vi "Consumer.vi"(8 "error in (no error)":errorcluster, 9 "Data":variant, 10 "Case ID":string, 11 "uService Template in":refnum<class "TCP Writer.lvclass">) -> (0 "error out":errorcluster, 3 "uService Template out":refnum<class "TCP Writer.lvclass">)   [LabVIEW 2020, in "TALOS.lvlib" / "TCP Writer.lvlib" / "TCP Writer.lvclass"]
uses:
  TCP Writer.lvclass
  C:/LabVIEW Code/TALOS/talos/Father of all uServices/Father of all uServices/Father of all uServices.lvclass
  TCP Writer Consumer Case Selector.ctl
  TCP Writer.lvclass/TCP Writer.ctl
  Father of all uServices/Father of all uServices Messages/Consumer Msg/Consumer Msg.lvclass/Consumer Msg.ctl
  Ancestor/Ancestor/Ancestor.lvclass/Ancestor.ctl
  Father of all uServices/Father of all uServices/Father of all uServices.lvclass/Father of all uServices.ctl
  Ancestor/Ancestor/Infinite Message Selector.ctl
  Support VIs/Generate Error.vi
  FGV/Error Memory/Get Error Description.vi
  Ancestor/Ancestor/Read ID.vi
  Support VIs/Get Class Name.vi
  FGV/Error Memory/Error Memory Core.vi
  <vilib>/AdvancedString/Delimited String to 1D String Array.vi
  Support VIs/Circus Root Path.vi
  FGV/Error Memory/Error Crt Lvl checker.vi
  FGV/Error Memory/Error Memory Core.vi/40c8088d-b597-4017-91af-faa98e00292e.vi
  FGV/Error Memory/Error Memory Core.vi/d4a3ab98-063c-4e44-b43d-fbdcfe6c2be2.vi
  Father of all uServices/Father of all uServices/Father of all uServices.lvclass
  C:/LabVIEW Code/TALOS/builds/Actor Framework PPL/Actor Framework.lvlibp/1abvi3w/vi.lib/ActorFramework/Actor/Actor.lvclass
  builds/Actor Framework PPL/Actor Framework.lvlibp/1abvi3w/vi.lib/ActorFramework/Actor/Read Self Enqueuer.vi
  <userlib>/_OpenG.lib/lvdata/lvdata.llb/Get Strings from Enum__ogtk.vi
  builds/Actor Framework PPL/Actor Framework.lvlibp/1abvi3w/vi.lib/ActorFramework/Message Enqueuer/Enqueue.vi
  Support VIs/Global Memory.vi
  Support VIs/Is in Packed Library.vi
  Support VIs/TALOS Root path.vi
  Support VIs/Read CSV worksheet.vi
  Support VIs/Global Constants.vi
  <vilib>/Utility/error.llb/General Error Handler.vi
  Support VIs/Error Log.vi
  Father of all uServices/Father of all uServices Messages/Consumer Msg/Consumer Msg.lvclass
  Ancestor/Ancestor/Ancestor.lvclass
  <vilib>/Comparison/Equal/Equal Functor/Equal Functor.lvclass
  TALOS.lvlib
  C:/LabVIEW Code/TALOS/talos/Ancestor/Ancestor/Ancestor.lvclass
  C:/LabVIEW Code/TALOS/talos/Internal uServices/System uServices/TCP Writer/TCP Writer/TCP Writer.lvclass
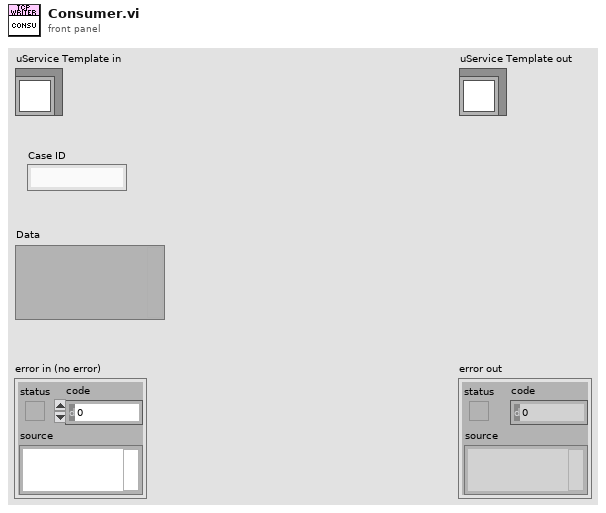
[diagram p1: front panel]
types:
  T1 = typedef "TALOS.lvlib/TCP Writer.lvlib/TCP Writer.lvclass/TCP Writer Consumer Case Selector.ctl" = enum16{"Send message", "Idle", "Check Connection", "Open connection", "Set Client ID"}
  T2 = typedef "TALOS.lvlib/Ancestor.lvlib/Ancestor.lvclass/Infinite Message Selector.ctl" = enum16{"Start", "Stop", "Check", "Flush (Stop all)", "Init"}
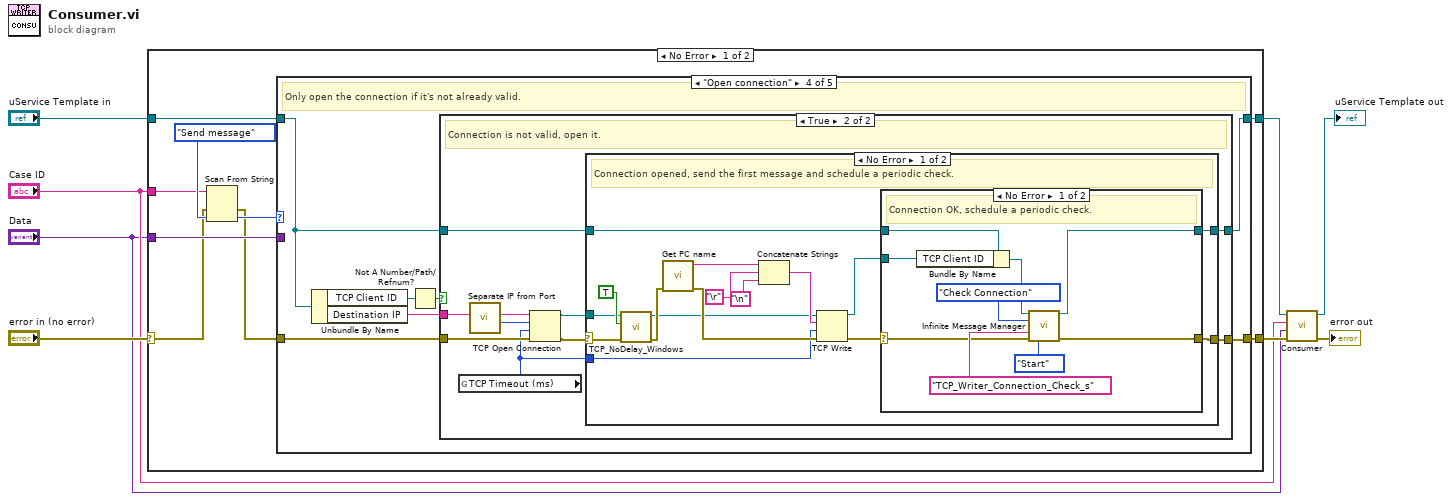
[diagram p0: block diagram]
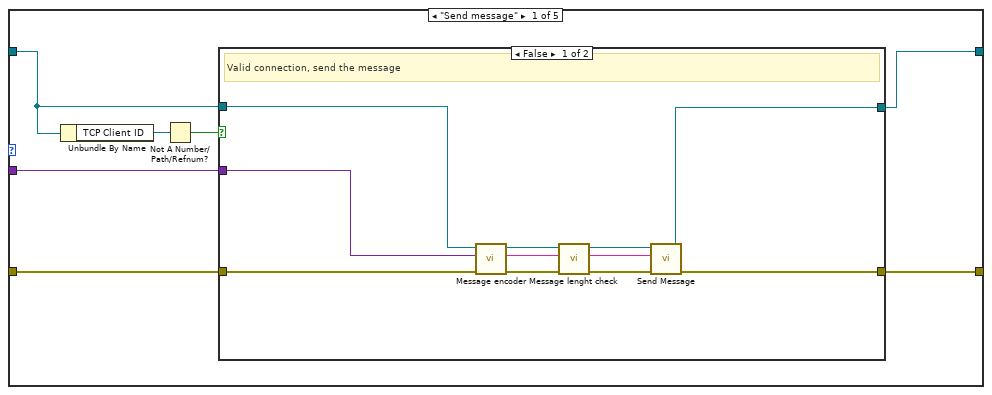
[diagram p2: hidden frame]
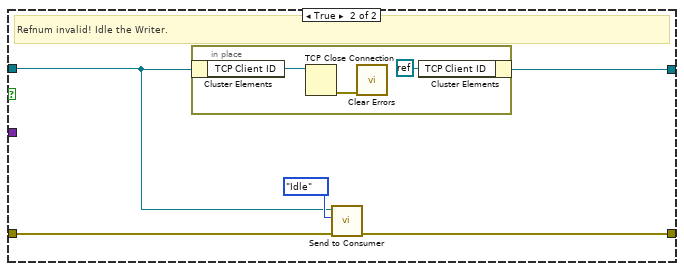
[diagram p3: hidden frame]
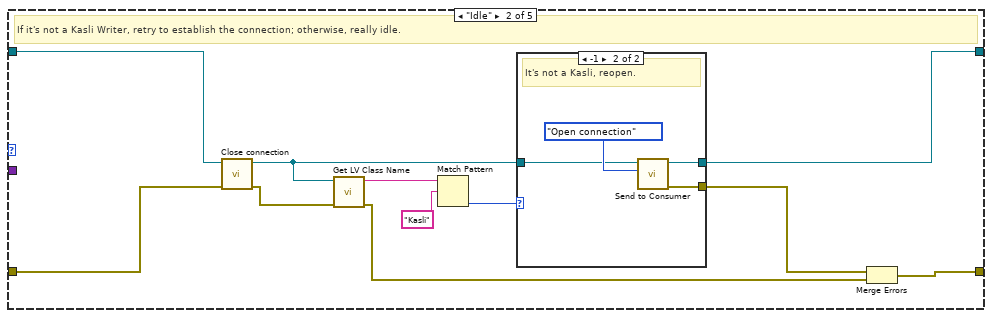
[diagram p4: hidden frame]
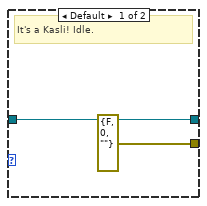
[diagram p5: hidden frame]
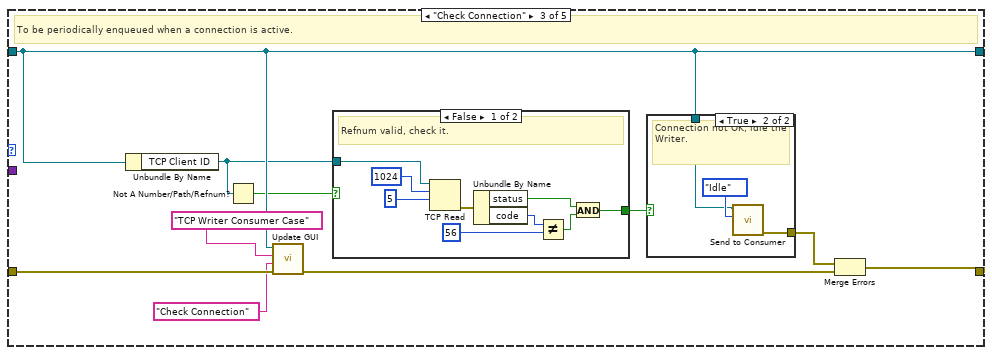
[diagram p6: hidden frame]
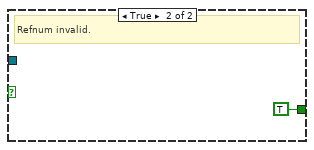
[diagram p7: hidden frame]
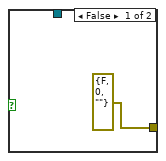
[diagram p8: hidden frame]
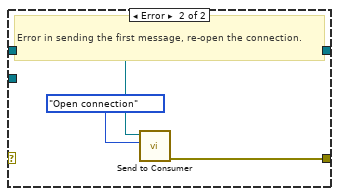
[diagram p10: hidden frame]
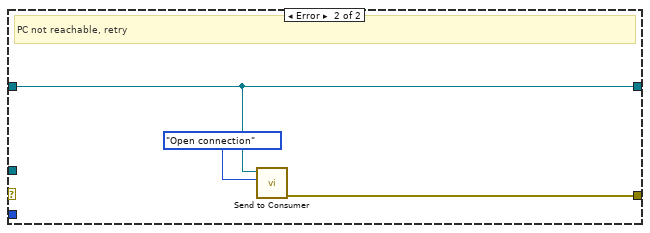
[diagram p11: hidden frame]
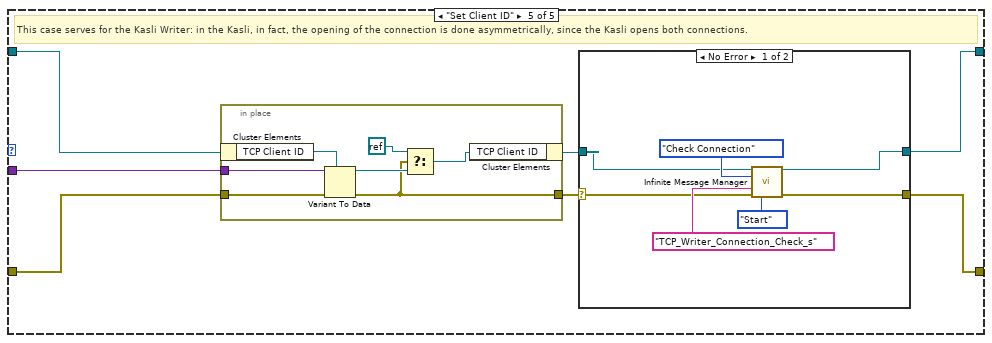
[diagram p12: hidden frame]
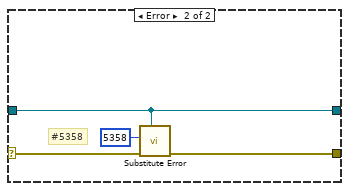
[diagram p13: hidden frame]
diagram:
  n1 = case shown="No Error" "error in (no error)" {
    selector: "error in (no error)" -> [w13 w160]
    tunnel: "uService Template in" -> [w12 w161]
    tunnel: [w15 w161] -> w4
    tunnel: [w16 w160] -> w3
    tunnel: "Case ID" -> [w10 _]
    tunnel: "Data" -> [w17 _]
    frame No Error {
      n2 = Scan From String(input string=w10, error in=w13, default 1=TCP_Writer_Consumer_Case_Selector."Send message") -> (error out=w9:errorcluster, output 1=w11:T1)  [unwired: 2 in, 2 out]
      n3 = case shown="\"Open connection\"" w11 {
        tunnel: w17 -> [w22 _ _ _ w137]
        tunnel: w9 -> [w21 w53 w65 w91 w136]
        tunnel: w12 -> [w23 w54 w66 w88 w139]
        tunnel: [w24 w50 w64 w89 w135] -> w16
        tunnel: [w18 w51 w66 w90 w138] -> w15
        frame "Send message" {
          n4 = Unbundle By Name(w23) -> ("TCP Client ID"=w20:refnum<k5>)
          n5 = Not A Number/Path/Refnum?(number/path/refnum=w20) -> (NaN/Path/Refnum?=w19:bool)
          n6 = case shown="False" w19 {
            tunnel: [w35 w38] -> w24
            tunnel: w23 -> [w34 w37]
            tunnel: w22 -> [w33 _]
            tunnel: w21 -> [w32 w39]
            tunnel: [w28 w36] -> w18
            frame False {
              # "Valid connection, send the message"
              n7 = call-dynamic "Message encoder.vi"("error in (no error)"=w32, "Data"=w33, "TCP Writer in"=w34) -> ("error out"=w31:errorcluster, "Message encoded"=w29:string, "TCP Writer out"=w30:refnum<class "TCP Writer.lvclass">)  [unwired: 6 in]
              n8 = call-dynamic "Message lenght check.vi"("error in (no error)"=w31, "String in"=w29, "TCP Writer in"=w30) -> ("error out"=w27:errorcluster, "String out"=w26:string, "TCP Writer out"=w25:refnum<class "TCP Writer.lvclass">)  [unwired: 6 in]
              n9 = call-dynamic "Send Message.vi"("error in (no error)"=w27, "String in"=w26, "TCP Writer in"=w25) -> ("error out"=w35:errorcluster, "TCP Writer out"=w28:refnum<class "TCP Writer.lvclass">)  [unwired: 7 in]
            }
            frame True {
              # "Refnum invalid! Idle the Writer."
              n10 = in-place {
                n11 = in-place-cluster #1(w37) -> ("TCP Client ID"=w43:refnum<k5>)
                n12 = TCP Close Connection(connection ID=w43) -> (error out=w42:errorcluster)  [unwired: 2 in, 1 out]
                n13 = call <vilib>:"Clear Errors.vi"("error in (no error)"=w42) -> ()  [unwired: 5 in, 2 out]
                n14 = in-place-cluster #1("TCP Client ID"=refnum<k0> refnum) -> (w36:refnum<class "TCP Writer.lvclass">)
              }
              n15 = call "Send to Consumer.vi"("error in (no error)"=w39, "Case ID"=TCP_Writer_Consumer_Case_Selector."Idle" ("TCP Listener Consumer Case Selector"), "uService Template in"=w37) -> ("error out"=w38:errorcluster)  [unwired: 7 in, 1 out]
            }
          }
        }
        frame "Idle" {
          # "If it's not a Kasli Writer, retry to establish the connection; otherwise, really idle."
          n16 = call-dynamic "Close connection.vi"("error in (no error)"=w53, "TCP Writer in"=w54) -> ("error out"=w45:errorcluster, "TCP Writer out"=w49:refnum<class "TCP Writer.lvclass">)  [unwired: 8 in]
          n17 = call <vilib>:"Get LV Class Name.vi"("error in (no error)"=w45, "object"=w49) -> ("error out"=w44:errorcluster, "class name"=w48:string)  [unwired: 8 in]
          n18 = Match Pattern(string=w48, regular expression="Kasli") -> (offset past match=w46:i32)  [unwired: 1 in, 3 out]
          n19 = case shown="-1" w46 {
            tunnel: w49 -> [w56 w59]
            tunnel: [errorcluster {"status"=FALSE, "code"=0, "source"=""} ("error out") w58] -> w52
            tunnel: [w56 w57] -> w51
            frame Default {
              # "It's a Kasli! Idle."
            }
            frame -1 {
              # "It's not a Kasli, reopen."
              n20 = call "Send to Consumer.vi"("Case ID"=TCP_Writer_Consumer_Case_Selector."Open connection" ("TCP Listener Consumer Case Selector"), "uService Template in"=w59) -> ("error out"=w58:errorcluster, "uService Template out"=w57:refnum<class "TCP Writer.lvclass">)  [unwired: 8 in]
            }
          }
          n21 = Merge Errors(w52, w44) -> (w50:errorcluster)
        }
        frame "Check Connection" {
          # "To be periodically enqueued when a connection is active."
          n22 = Unbundle By Name(w66) -> ("TCP Client ID"=w62:refnum<k5>)
          n23 = Not A Number/Path/Refnum?(number/path/refnum=w62) -> (NaN/Path/Refnum?=w63:bool)
          n24 = call "Update GUI.vi"("error in (no error)"=w65, "Data"="Check Connection", "GUI Item Name"="TCP Writer Consumer Case", "uService Template in"=w66) -> ("error out"=w69:errorcluster)  [unwired: 6 in, 1 out]
          n25 = case shown="False" w63 {
            tunnel: w62 -> [w79 _]
            tunnel: [w74 TRUE] -> w70
            frame False {
              # "Refnum valid, check it."
              n26 = TCP Read(connection ID=w79, bytes to read=1024, 9:5 ("timeout ms (25000)")) -> (error out=w78:errorcluster)  [unwired: 2 in, 2 out]
              n27 = Unbundle By Name(w78) -> ("status"=w75:bool, "code"=w77:i32)
              n28 = Not Equal?(x=w77, y=56) -> (x != y?=w76:bool)
              n29 = And(x=w75, y=w76) -> (x .and. y?=w74:bool)
            }
            frame True {
              # "Refnum invalid."
            }
          }
          n30 = case shown="True" w70 {
            tunnel: w66 -> [_ w83]
            tunnel: [errorcluster {"status"=FALSE, "code"=0, "source"=""} ("error out") w82] -> w68
            frame False {
            }
            frame True {
              # "Connection not OK, idle the Writer."
              n31 = call "Send to Consumer.vi"("Case ID"=TCP_Writer_Consumer_Case_Selector."Idle" ("TCP Listener Consumer Case Selector"), "uService Template in"=w83) -> ("error out"=w82:errorcluster)  [unwired: 8 in, 1 out]
            }
          }
          n32 = Merge Errors(w68, w69) -> (w64:errorcluster)
        }
        frame "Open connection" {
          # "Only open the connection if it's not already valid."
          n33 = Unbundle By Name(w88) -> ("TCP Client ID"=w87:refnum<k5>, "Destination IP"=w85:string)
          n34 = Not A Number/Path/Refnum?(number/path/refnum=w87) -> (NaN/Path/Refnum?=w86:bool)
          n35 = case shown="True" w86 {
            tunnel: w91 -> [w92 w103]
            tunnel: w88 -> [w93 w102]
            tunnel: [w93 w101] -> w90
            tunnel: [w92 w100] -> w89
            tunnel: w85 -> [_ w96]
            frame False {
              # "Connection is already valid, do not open it!"
            }
            frame True {
              # "Connection is not valid, open it."
              n36 = global read "Global Constants.vi" "TCP Timeout (ms)"() -> (w99:i32)
              n37 = call "Separate IP from Port.vi"("IP+Port"=w96) -> ("Port"=w94:u16, "IP"=w95:string)  [unwired: 9 in]
              n38 = TCP Open Connection(address=w95, remote port or service name=w94, timeout ms (60000)=w99, error in (no error)=w103) -> (connection ID=w98:refnum<k5>, error out=w97:errorcluster)  [unwired: 1 in]
              n39 = case shown="No Error" w97 {
                selector: w97 -> [w107 _]
                tunnel: w98 -> [w105 _]
                tunnel: w102 -> [w119 w132]
                tunnel: [w118 w132] -> w101
                tunnel: [w117 w133] -> w100
                tunnel: w99 -> [w109 _]
                frame No Error {
                  # "Connection opened, send the first message and schedule a periodic check."
                  n40 = call "TCP_NoDelay_Windows.vi"("error in (no error)"=w107, "TCP_NODELAY (true)"=TRUE, "connID"=w105) -> ("error out"=w106:errorcluster, "connID 2"=w104:refnum<k5>)  [unwired: 3 in]
                  n41 = call "Get PC name.vi"("error in (no error)"=w106) -> ("error out"=w111:errorcluster, "Hostname"=w110:string)  [unwired: 9 in]
                  n42 = Concatenate Strings(w110, "\r", "\n") -> (w112:string)
                  n43 = TCP Write(connection ID=w104, data in=w112, error in (no error)=w111, 9:w109) -> (connection ID out=w116:refnum<k5>, error out=w115:errorcluster)  [unwired: 1 out]
                  n44 = case shown="No Error" w115 {
                    selector: w115 -> [w121 _]
                    tunnel: w119 -> [w128 w129]
                    tunnel: [w124 w129] -> w118
                    tunnel: [w123 w130] -> w117
                    tunnel: w116 -> [w122 _]
                    frame No Error {
                      # "Connection OK, schedule a periodic check."
                      n45 = Bundle By Name(cluster=w128, "TCP Client ID"=w122) -> (w125:refnum<class "TCP Writer.lvclass">)
                      n46 = call-dynamic "Infinite Message Manager.vi"("Father of all uServices in"=w125, "Consumer Case Selector"=TCP_Writer_Consumer_Case_Selector."Check Connection", "Tau parameter"="TCP_Writer_Connection_Check_s", "error in (no error)"=w121, "Infinite Message Selector"=Infinite_Message_Selector."Start") -> ("Father of all uServices out"=w124:refnum<class "TCP Writer.lvclass">, "error out"=w123:errorcluster)  [unwired: 8 in, 1 out]
                    }
                    frame Error {
                      # "Error in sending the first message, re-open the connection."
                      n47 = call "Send to Consumer.vi"("Case ID"=TCP_Writer_Consumer_Case_Selector."Open connection" ("TCP Listener Consumer Case Selector"), "uService Template in"=w129) -> ("error out"=w130:errorcluster)  [unwired: 8 in, 1 out]
                    }
                  }
                }
                frame Error {
                  # "PC not reachable, retry"
                  n48 = call "Send to Consumer.vi"("Case ID"=TCP_Writer_Consumer_Case_Selector."Open connection" ("TCP Listener Consumer Case Selector"), "uService Template in"=w132) -> ("error out"=w133:errorcluster)  [unwired: 8 in, 1 out]
                }
              }
            }
          }
        }
        frame "Set Client ID" {
          # "This case serves for the Kasli Writer: in the Kasli, in fact, the opening of the connection is done asymmetrically, since the Kasli opens both connections."
          n49 = in-place "In Place Element Structure" {
            in-place-border: w137 -> [w159]
            in-place-border: w136 -> [w158]
            in-place-border: [w154] -> w141
            n50 = in-place-cluster #2(w139) -> ("TCP Client ID"=w155:refnum<k5>)
            n51 = Variant To Data(error in=w158, type=w155, Variant=w159) -> (data=w157:refnum<k5>, error out=w154:errorcluster)
            n52 = Select(t=refnum<k0> refnum, s=w154, f=w157) -> (s? t:f=w156:refnum<k5>)
            n53 = in-place-cluster #2("TCP Client ID"=w156) -> (w140:refnum<class "TCP Writer.lvclass">)
          }
          n54 = case shown="No Error" w141 {
            selector: w141 -> [w145 w151]
            tunnel: [w144 w150] -> w135
            tunnel: w140 -> [w143 w149]
            tunnel: [w142 w149] -> w138
            frame No Error {
              n55 = call-dynamic "Infinite Message Manager.vi"("Father of all uServices in"=w143, "Consumer Case Selector"=TCP_Writer_Consumer_Case_Selector."Check Connection", "Tau parameter"="TCP_Writer_Connection_Check_s", "error in (no error)"=w145, "Infinite Message Selector"=Infinite_Message_Selector."Start") -> ("Father of all uServices out"=w142:refnum<class "TCP Writer.lvclass">, "error out"=w144:errorcluster)  [unwired: 8 in, 1 out]
            }
            frame Error {
              # "#5358"
              n56 = call "Substitute Error.vi"("LabVIEW Object"=w149, "error in (no error)"=w151, "Error Code"=5358) -> ("error out"=w150:errorcluster)  [unwired: 8 in]
            }
          }
        }
      }
    }
    frame Error {
    }
  }
  n57 = call-parent "Consumer.vi"("error in (no error)"=w3, "Data"="Data", "Case ID"="Case ID", "uService Template in"=w4) -> ("error out"=→"error out":errorcluster, "uService Template out"=→"uService Template out":refnum<class "TCP Writer.lvclass">)  [unwired: 6 in]
